vi "RemoteVI Add Client.vi"(0 "connection":u32, 1 "hWnd":u64, 2 "address":string, 3 "view only?":bool, 5 "clients":T1(array[cluster]), 7 "hello":string, 9 "overlay frame":string) -> (4 "clients out":T1(array[cluster]))   [LabVIEW 2020, in "RemoteVI.lvlib"]
doc: "Greets a freshly upgraded WebSocket connection and appends it to clients (with its peer address, connected since now and view only): restores a minimized panel (RemoteVI Restore If Minimized.vi on hWnd), writes hello (the title and viewonly text messages) followed by overlay frame (the current OVERLAY, empty when no popup is open) with a 2 s timeout, and appends a new client with that connection; closed is set when the write failed. connection is the TCP connection refnum type-cast to U32."
uses:
  RemoteVI.lvlib
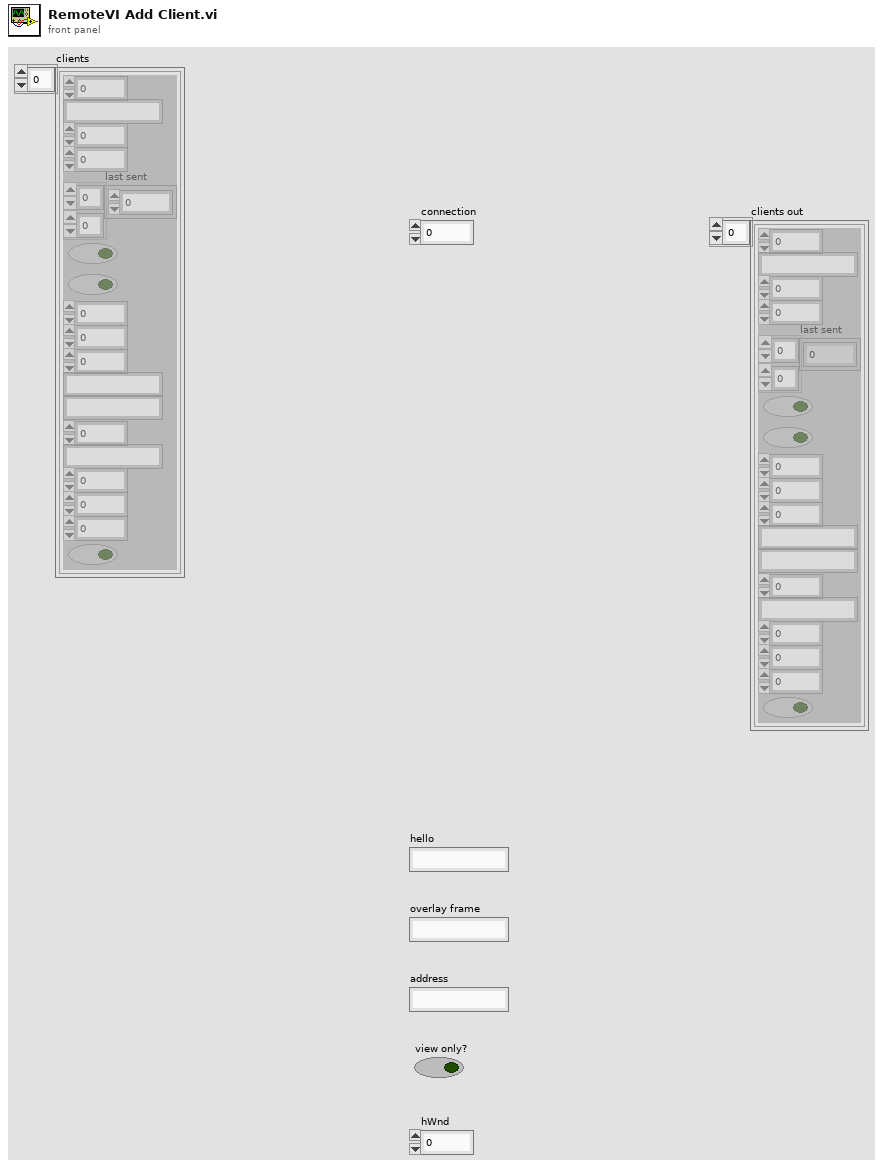
[diagram p1: front panel]
types:
  T1 = cluster{"connection":u32, "rx buffer":string, "seq":u32, "acked":u32, "last sent":u32[][], "tracking":bool, "closed":bool, "mods":u8, "mods set":u8, "popup since":u32, "windows sent":string, "window frames":cluster{"id":u64, "pixels":u32[][]}[], "key window":u64, "address":string, "since":dbl, "last input":dbl, "bytes":dbl, "view only":bool}[]
  T2 = cluster{"connection":u32, "rx buffer":string, "seq":u32, "acked":u32, "last sent":u32[][], "tracking":bool, "closed":bool, "mods":u8, "mods set":u8, "popup since":u32, "windows sent":string, "window frames":cluster{"id":u64, "pixels":u32[][]}[], "key window":u64, "address":string, "since":dbl, "last input":dbl, "bytes":dbl, "view only":bool}
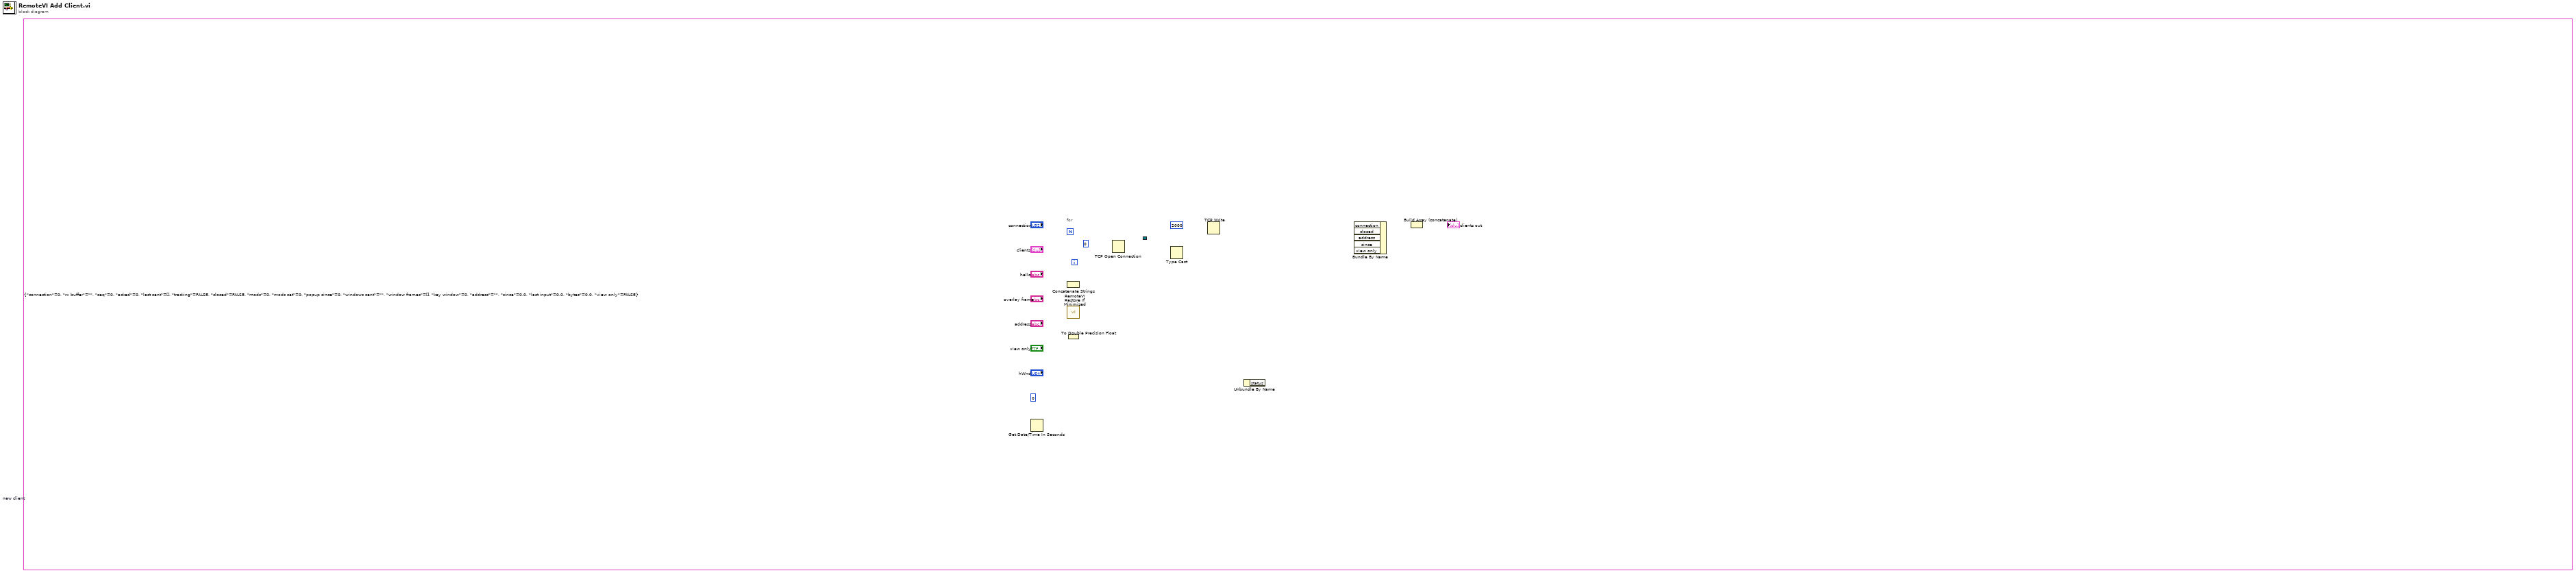
[diagram p0: block diagram]
diagram:
  w15 = T2 {"connection"=0, "rx buffer"="", "seq"=0, "acked"=0, "last sent"=[], "tracking"=FALSE, "closed"=FALSE, "mods"=0, "mods set"=0, "popup since"=0, "windows sent"="", "window frames"=[], "key window"=0, "address"="", "since"=0.0, "last input"=0.0, "bytes"=0.0, "view only"=FALSE}  # new client
  n1 = Get Date/Time In Seconds() -> (seconds since 1Jan1904=w16:timestamp)
  n2 = for {
    N: 0 -> [_]
    tunnel: [w21] -> w9
    # "Never runs: TCP refnum type only"
    n3 = TCP Open Connection(remote port or service name=u16 0) -> (connection ID=w21:refnum<k5>)  [unwired: 4 in, 1 out]
  }
  n4 = Concatenate Strings("hello", "overlay frame") -> (w11:string)
  n5 = call "RemoteVI Restore If Minimized.vi"("hWnd"="hWnd") -> ()  [unwired: 13 in, 2 out]
  n6 = To Double Precision Float(number=w16) -> (double precision float=w17:dbl)
  n7 = Type Cast(type=w9, x="connection") -> (*(type *) &x=w10:refnum<k5>)
  n8 = TCP Write(connection ID=w10, data in=w11, 9:2000) -> (error out=w13:errorcluster)  [unwired: 1 in, 2 out]
  n9 = Unbundle By Name(w13) -> ("status"=w14:bool)
  n10 = Bundle By Name(cluster=w15, "connection"="connection", "closed"=w14, "address"="address", "since"=w17, "view only"="view only?") -> (w18:T2)
  n11 = Build Array (concatenate)("clients", w18) -> (→"clients out":T1)
